vi "layout.vi"(0 "reference":refnum<class "ImplicitParameterNode.lvclass">, 1 "graph":refnum<class "Graph.lvclass">, 2 "graphics":refnum<class "Graphics.lvclass">, 3 "grid":refnum<class "Grid.lvclass">, 5 "error in (no error)":errorcluster) -> (14 "reference out":refnum<class "ImplicitParameterNode.lvclass">, 19 "error out":errorcluster)   [LabVIEW 2020, in "ImplicitParameterNode.lvclass"]
doc: "public void layout(Graph g, Graphics2D g2, Grid grid)"
uses:
  <resource>/Framework/Providers/Open_GDS/UML/ImplicitParameterNode_class/ImplicitParameterNode.lvclass
  C:/Program Files (x86)/National Instruments/LabVIEW 2020/resource/Framework/Providers/Open_GDS/UML/RectangularNode_class/RectangularNode.lvclass
  <resource>/Framework/Providers/Open_GDS/UML/Graph_class/Graph.lvclass
  <resource>/Framework/Providers/Open_GDS/UML/Graphics_class/Graphics.lvclass
  <resource>/Framework/Providers/Open_GDS/UML/Grid_class/Grid.lvclass
  <resource>/Framework/Providers/Open_GDS/UML/General/Rectangle/Rectangle Rectangle2D.ctl
  <resource>/Framework/Providers/Open_GDS/UML/MultiLineString_class/MultiLineString.lvclass
  <resource>/Framework/Providers/Open_GDS/UML/RectangularNode_class/RectangularNode.lvclass
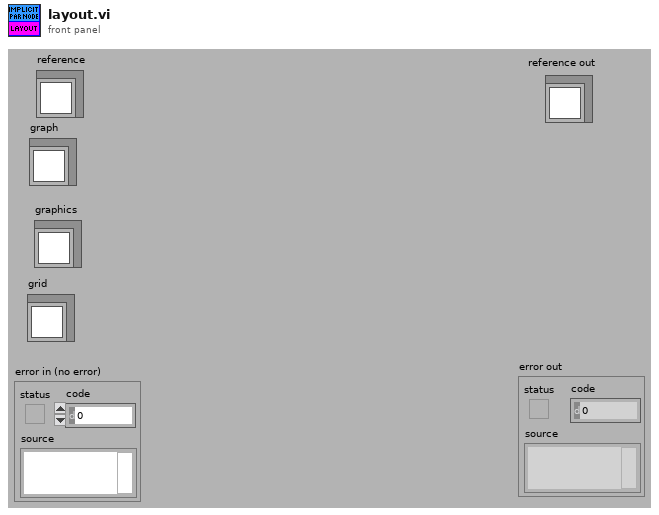
[diagram p1: front panel]
types:
  T1 = typedef "Rectangle Rectangle2D.ctl" = cluster{"x":dbl, "y":dbl, "width":dbl, "height":dbl}
  T2 = typedef "ImplicitParameterNode.lvclass/ObjectAttributes.ctl" = cluster{"topHeight":dbl, "name":refnum<class "MultiLineString.lvclass">, "DEFAULT_TOP_HEIGHT":i32, "DEFAULT_WIDTH":i32, "DEFAULT_HEIGHT":i32}
  T3 = typedef "RectangularNode.lvclass/ObjectAttributes.ctl" = cluster{"bounds":T1}
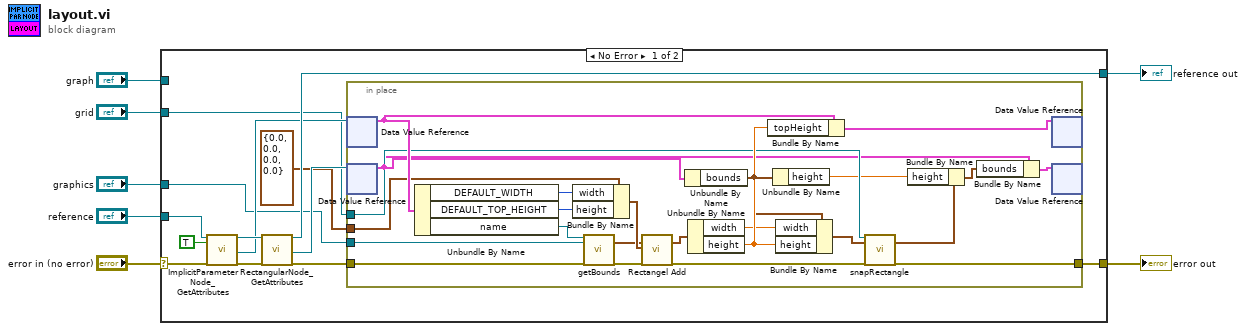
[diagram p0: block diagram]
diagram:
  n1 = case shown="No Error" "error in (no error)" {
    selector: "error in (no error)" -> [w17 w45]
    tunnel: "reference" -> [w20 w46]
    tunnel: [w19 w45] -> w6
    tunnel: [w18 w46] -> w5
    tunnel: "graphics" -> [w10 _]
    tunnel: "grid" -> [w8 _]
    tunnel: "graph" -> [_ _]
    frame No Error {
      n2 = call <resource>:"ImplicitParameterNode_GetAttributes.vi"("reference in"=w20, "OnlyGetDvrReference(False)"=TRUE, "error in (no error)"=w17) -> ("reference out"=w15:refnum<class "ImplicitParameterNode.lvclass">, "DataRef"=w13:refnum<data-value>, "error out"=w14:errorcluster)  [unwired: 13 in, 1 out]
      n3 = call <resource>:"RectangularNode_GetAttributes.vi"("reference in"=w15, "error in (no error)"=w14) -> ("reference out"=w18:refnum<class "ImplicitParameterNode.lvclass">, "DataRef"=w12:refnum<data-value>, "error out"=w9:errorcluster)  [unwired: 14 in, 1 out]
      n4 = in-place {
        in-place-border: T1 {"x"=0.0, "y"=0.0, "width"=0.0, "height"=0.0} ("bounds") -> [w34]
        in-place-border: w10 -> [w32]
        in-place-border: w9 -> [w31]
        in-place-border: w8 -> [w27]
        in-place-border: [w25] -> w19
        n5 = in-place-dvr #1(w13) -> (w44:T2)  [unwired: 1 out]
        n6 = in-place-dvr #2(w12) -> (w24:T3)  [unwired: 1 out]
        n7 = Unbundle By Name(w44) -> ("DEFAULT_WIDTH"=w41:i32, "DEFAULT_TOP_HEIGHT"=w40:i32, "name"=w39:refnum<class "MultiLineString.lvclass">)
        n8 = Bundle By Name(cluster=w34, "width"=w41, "height"=w40) -> (w33:T1)
        n9 = call-dynamic "getBounds.vi"("reference"=w39, "graphics"=w32, "error in (no error)"=w31) -> ("bounds"=w30:T1, "error out"=w29:errorcluster)  [unwired: 15 out]
        n10 = call <resource>:"Rectangel Add.vi"("bounds1"=w30, "bounds2"=w33, "error in (no error)"=w29) -> ("boundsAdded"=w38:T1, "error out"=w28:errorcluster)  [unwired: 2 in, 13 out]
        n11 = Unbundle By Name(w24) -> ("bounds"=w36:T1)
        n12 = Unbundle By Name(w38) -> ("width"=w37:dbl, "height"=w43:dbl)
        n13 = Bundle By Name(cluster=w44, "topHeight"=w43) -> (w42:T2)
        n14 = Unbundle By Name(w36) -> ("height"=w23:dbl)
        n15 = Bundle By Name(cluster=w36, "width"=w37, "height"=w43) -> (w35:T1)
        n16 = call <resource>:"snapRectangle.vi"("reference"=w27, "bounds"=w35, "error in (no error)"=w28) -> ("boundsOut"=w26:T1, "error out"=w25:errorcluster)  [unwired: 15 out]
        n17 = Bundle By Name(cluster=w26, "height"=w23) -> (w22:T1)
        n18 = Bundle By Name(cluster=w24, "bounds"=w22) -> (w21:T3)
        n19 = in-place-dvr #1(w42) -> ()  [unwired: 2 out]
        n20 = in-place-dvr #2(w21) -> ()  [unwired: 2 out]
      }
    }
    frame Error {
    }
  }
  "reference out" <- w5
  "error out" <- w6
